vi "Move TurnTable.vi"(8 "error in (no error)":errorcluster caption="에러 입력(에러 없음)", 10 "Turn Table Info":T1, 11 "Instrument Manager 입력":refnum<class "Instrument Manager.lvclass">) -> (0 "error out":errorcluster caption="에러 출력", 3 "Instrument Manager 출력":refnum<class "Instrument Manager.lvclass">)   [LabVIEW 2023, in "Instrument Manager.lvclass"]
uses:
  Instrument Manager.lvclass
  Instrument Manager.lvclass/Instrument Manager.ctl
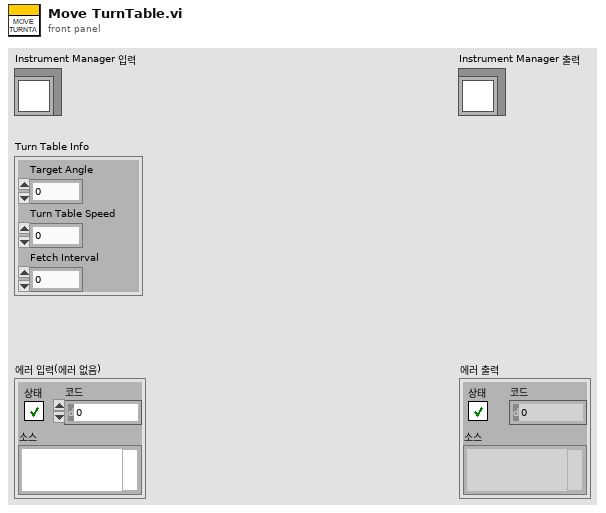
[diagram p1: front panel]
types:
  T1 = cluster{"Target Angle":dbl, "Turn Table Speed":i32, "Fetch Interval":i32}
  T2 = cluster{"Turn Table Info":cluster{"Target Angle":dbl, "Turn Table Speed":i32, "Fetch Interval":i32}, "Instrument Manager 입력":refnum<class "Instrument Manager.lvclass">}
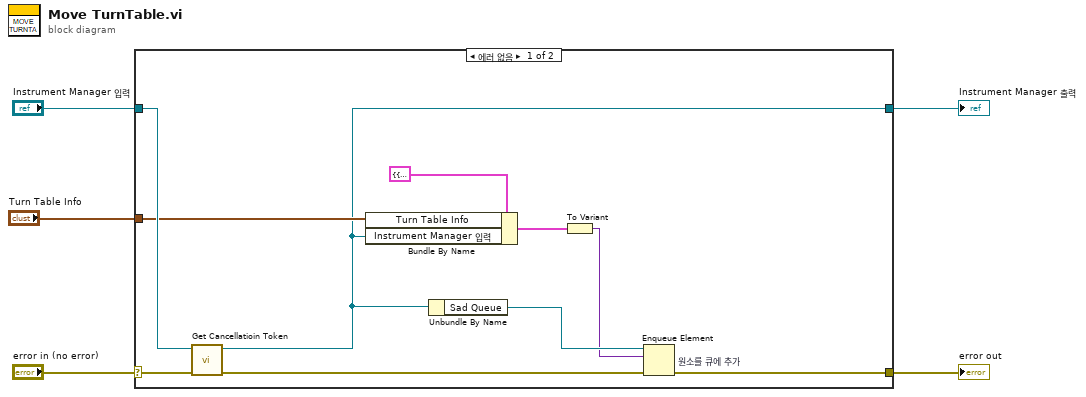
[diagram p0: block diagram]
diagram:
  n1 = case shown="에러 없음" "error in (no error)" {
    selector: "error in (no error)" -> [w15 w17]
    tunnel: [w7 w17] -> w4
    tunnel: [w6 w16] -> w2
    tunnel: "Instrument Manager 입력" -> [w14 w16]
    tunnel: "Turn Table Info" -> [w12 _]
    frame No Error {
      n2 = call "Get Cancellatioin Token.vi"("error in (no error)"=w15, "Instrument Manager 입력"=w14) -> ("error out"=w8:errorcluster, "Instrument Manager 출력"=w6:refnum<class "Instrument Manager.lvclass">)  [unwired: 7 in, 1 out]
      n3 = Bundle By Name(cluster=T2 {"Turn Table Info"={"Target Angle"=0.0, "Turn Table Speed"=0, "Fetch Interval"=0}, "Instrument Manager 입력"=refnum} ("원소"), "Turn Table Info"=w12, "Instrument Manager 입력"=w6) -> (w10:T2)
      n4 = Unbundle By Name(w6) -> ("Sad Queue"=w11:refnum<queue>)
      n5 = To Variant(anything=w10) -> (Variant=w9:variant)
      n6 = Enqueue Element "원소를 큐에 추가"(queue=w11, element=w9, error in (no error)=w8) -> (error out=w7:errorcluster)  [unwired: 1 in, 2 out]
    }
    frame Error {
    }
  }
  "error out" <- w4
  "Instrument Manager 출력" <- w2
